vi "get_profile_details.vi"(8 "error in (no error)":errorcluster, 11 "path":path) -> (0 "error out":errorcluster, 3 "standard output":string)   [LabVIEW 2021]
panel:
  out "concatenated string":string
  out "standard error":string
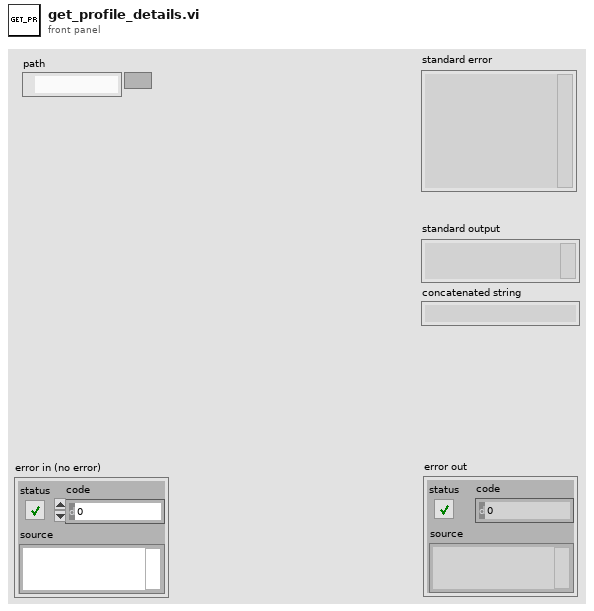
[diagram p1: front panel]
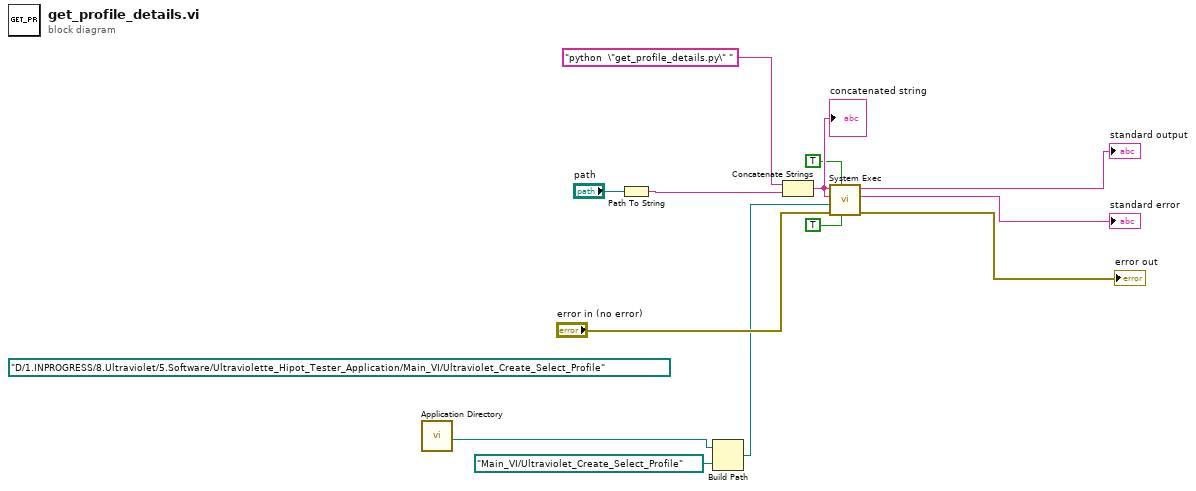
[diagram p0: block diagram]
diagram:
  (unwired) path "D:/1.INPROGRESS/8.Ultraviolet/5.Software/Ultraviolette_Hipot_Tester_Application/Main_VI/Ultraviolet_Create_Select_Profile" ("working directory")
  n1 = call <vilib>:"Application Directory.vi"() -> ("Application Directory"=w4:path)
  n2 = Path To String(path="path") -> (string=w3:string)
  n3 = Build Path(base path=w4, name or relative path=path "Main_VI/Ultraviolet_Create_Select_Profile") -> (appended path=w1:path)
  n4 = Concatenate Strings("python  \"get_profile_details.py\" " ("command line"), w3) -> (w11:string)
  "concatenated string" <- w11
  n5 = call <vilib>:"System Exec.vi"("run minimized? (F)"=TRUE, "wait until completion? (T)"=TRUE, "error in (no error)"="error in (no error)", "working directory"=w1, "standard input"=w11, "command line"=w11) -> ("error out"=→"error out":errorcluster, "standard error"=→"standard error":string, "standard output"=→"standard output":string)  [unwired: 2 in, 1 out]
